vi "Load SA Level Setting.vi"(8 "error in (no error)":errorcluster caption="에러 입력(에러 없음)", 10 "SA Level Param":T1, 11 "Instrument Manager 입력":refnum<class "Instrument Manager.lvclass">) -> (0 "error out":errorcluster caption="에러 출력", 3 "Instrument Manager 출력":refnum<class "Instrument Manager.lvclass">)   [LabVIEW 2023, in "Instrument Manager.lvclass"]
uses:
  Instrument Manager.lvclass
  Instrument Manager.lvclass/Instrument Manager.ctl
  Type Definition/SA Level Param.ctl
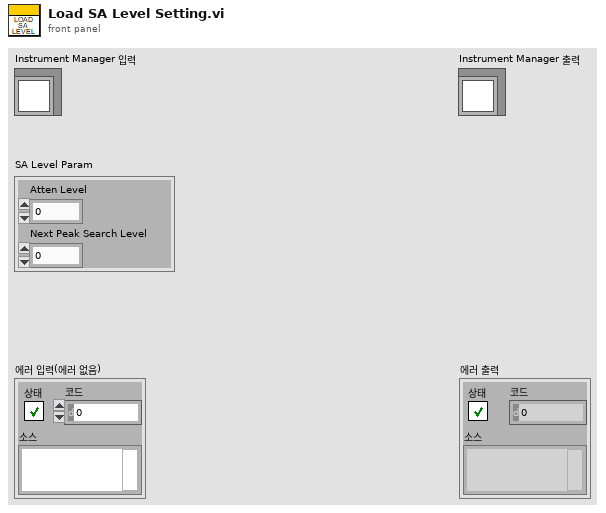
[diagram p1: front panel]
types:
  T1 = typedef "SA Level Param.ctl" = cluster{"Atten Level":dbl, "Next Peak Search Level":dbl}
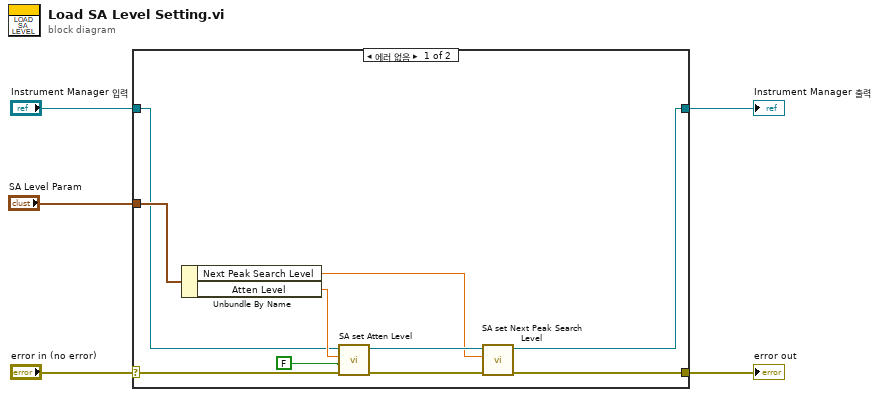
[diagram p0: block diagram]
diagram:
  n1 = case shown="에러 없음" "error in (no error)" {
    selector: "error in (no error)" -> [w14 w17]
    tunnel: [w12 w17] -> w4
    tunnel: [w8 w16] -> w2
    tunnel: "Instrument Manager 입력" -> [w10 w16]
    tunnel: "SA Level Param" -> [w15 _]
    frame No Error {
      n2 = Unbundle By Name(w15) -> ("Next Peak Search Level"=w6:dbl, "Atten Level"=w11:dbl)
      n3 = call "SA set Atten Level.vi"("error in (no error)"=w14, "Auto?"=FALSE, "Attenuation"=w11, "Instrument Manager 입력"=w10) -> ("error out"=w13:errorcluster, "Instrument Manager 출력"=w9:refnum<class "Instrument Manager.lvclass">)  [unwired: 6 in]
      n4 = call "SA set Next Peak Search Level.vi"("error in (no error)"=w13, "Peak Excursion"=w6, "Instrument Manager 입력"=w9) -> ("error out"=w12:errorcluster, "Instrument Manager 출력"=w8:refnum<class "Instrument Manager.lvclass">)  [unwired: 7 in]
    }
    frame Error {
    }
  }
  "error out" <- w4
  "Instrument Manager 출력" <- w2
